vi "SetChannel.vi"() -> ()   [LabVIEW 2015]
panel:
  in  "VISA资源名称":refnum<visa-resource-name>
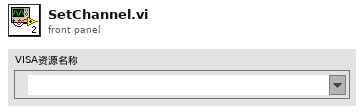
[diagram p1: front panel]
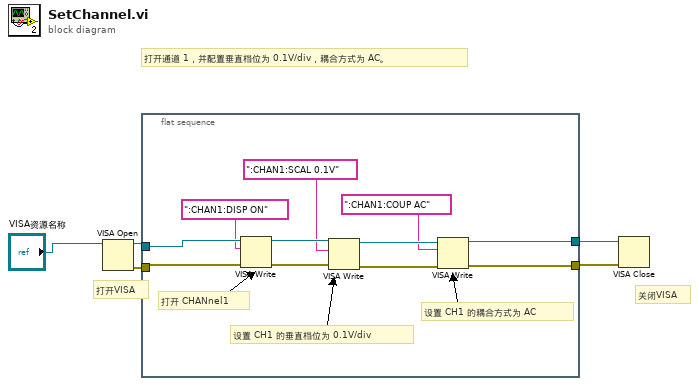
[diagram p0: block diagram]
diagram:
  # "关闭VISA"
  # "打开VISA"
  # "打开通道 1，并配置垂直档位为 0.1V/div，耦合方式为 AC。"
  n1 = VISA Open(VISA resource name="VISA资源名称") -> (VISA resource name=w5:refnum<visa-resource-name>, error out=w4:errorcluster)  [unwired: 4 in]
  n2 = flat-sequence {
    tunnel: w5 -> [w16]
    tunnel: w4 -> [w15]
    tunnel: [w11] -> w2
    tunnel: [w8] -> w1
    frame #0 {
      # "设置 CH1 的耦合方式为 AC"
      # "设置 CH1 的垂直档位为 0.1V/div"
      # "打开 CHANnel1"
      n3 = VISA Write(VISA resource name=w16, write buffer=":CHAN1:DISP ON", error in (no error)=w15) -> (VISA resource name out=w13:refnum<visa-resource-name>, error out=w10:errorcluster)  [unwired: 1 out]
      n4 = VISA Write(VISA resource name=w13, write buffer=":CHAN1:SCAL 0.1V" ("写入缓冲区"), error in (no error)=w10) -> (VISA resource name out=w12:refnum<visa-resource-name>, error out=w9:errorcluster)  [unwired: 1 out]
      n5 = VISA Write(VISA resource name=w12, write buffer=":CHAN1:COUP AC" ("写入缓冲区"), error in (no error)=w9) -> (VISA resource name out=w11:refnum<visa-resource-name>, error out=w8:errorcluster)  [unwired: 1 out]
    }
  }
  n6 = VISA Close(VISA resource name=w2, error in (no error)=w1) -> ()  [unwired: 1 out]
